vi "parse tdms properties_extract_priv_method.vi"(10 "property names":string[](array[string]), 11 "property values":variant[](array[variant])) -> (2 "channel units":string, 3 "nominal-compatible properties":map{string, string}(c390))   [LabVIEW 2020, in "Nominal-TDMS-Upload.lvlib" / "Nominal-TDMS-Upload.lvclass"]
uses:
  Nominal-TDMS-Upload.lvclass
  <vilib>/Nominal/Nominal IO Client/lv_src/Nominal Client/Nominal Client.lvclass
  <vilib>/Utility/Data Type/NI_Data Type.lvlib
  bb066b67-f704-4680-a74d-5f147d6b3788.vi
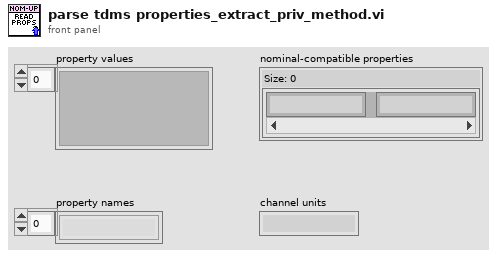
[diagram p1: front panel]
types:
  T1 = typedef "NI_Data Type.lvlib/Data Type.ctl" = enum8{"Invalid Type", "Void", "I8", "I16", "I32", "I64", "U8", "U16", "U32", "U64", "Single Float", "Double Float", "Extended Float", "Single Complex", "Double Complex", "Extended Complex", "Enum U8", "Enum U16", "Enum U32", "Enum U64", "Single Float With Unit", "Double Float With Unit", "Extended Float With Unit", "Single Complex with Unit", "Double Complex with Unit", "Extended Complex with Unit", "Boolean", "String", "Path", "Picture", "Tag", "Array", "Cluster", "Variant", "LV Variant", "Waveform", "Timestamp", "Digital Waveform", "Digital Data", "ExpressData", "Refnum", "External Data", "VI", "Poly VI", "LabVIEW Class Instance", "Fixed Point", "Set Collection", "Map Collection"}
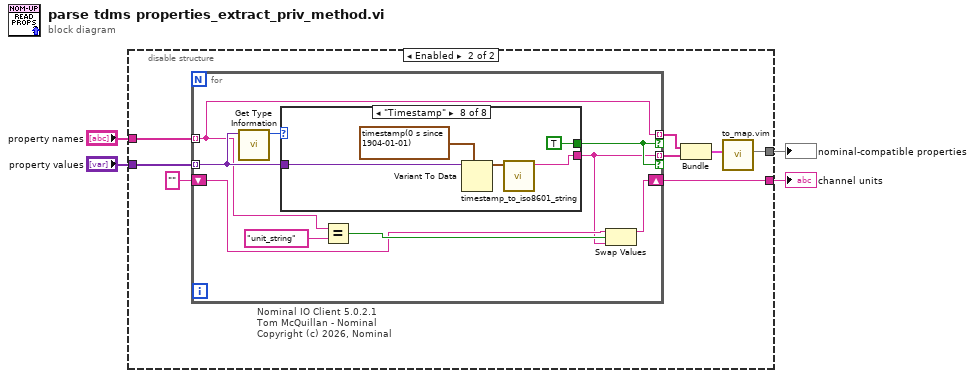
[diagram p0: block diagram]
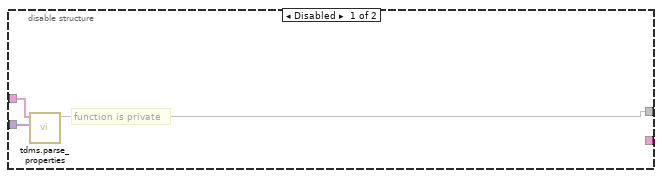
[diagram p2: hidden frame]
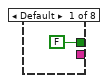
[diagram p3: hidden frame]
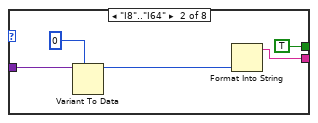
[diagram p4: hidden frame]
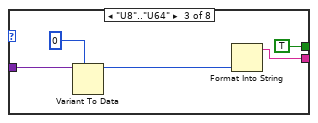
[diagram p5: hidden frame]
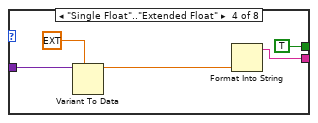
[diagram p6: hidden frame]
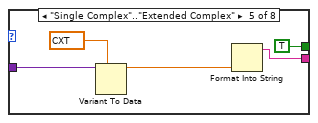
[diagram p7: hidden frame]
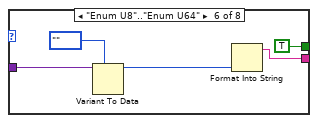
[diagram p8: hidden frame]
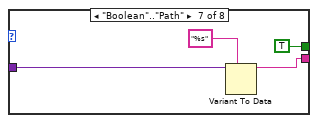
[diagram p9: hidden frame]
diagram:
  n1 = disable-structure shown="Enabled" {
    disable-tunnel: [w7 w10] -> w1
    disable-tunnel: "property names" -> [w6 w11]
    disable-tunnel: "property values" -> [w5 w12]
    disable-tunnel: [_ w8] -> w4
    frame Disabled {
      # "function is private"
      n2 = call <vilib>:"tdms.parse_properties.vi"("Property Values"=w5, "Property Names"=w6) -> ("Property Map"=w7:map{string, string})  [unwired: 9 in]
    }
    frame Enabled {
      # "Nominal IO Client 5.0.2.1\nTom McQuillan - Nominal\nCopyright (c) 2026, Nominal"
      n3 = for {
        tunnel: w12 -> [w23] mode=indexing
        tunnel: [w16] -> w15 mode=indexing if=w22
        tunnel: w11 -> [w21] mode=indexing
        tunnel: [w21] -> w14 mode=indexing if=w22
        shift-right: [w17] -> w8
        shift-left: "" -> [w18]
        n4 = call <vilib>:"Get Type Information.vi"("variant"=w23) -> ("type"=w24:T1)  [unwired: 6 in, 4 out]
        n5 = case shown="\"Timestamp\"" w24 {
          tunnel: w23 -> [_ w30 w35 w38 w43 w49 w54 w59]
          tunnel: [_ w27 w32 w37 w42 w47 w52 w55] -> w16
          tunnel: [FALSE TRUE TRUE TRUE TRUE TRUE TRUE TRUE] -> w22
          frame Default {
          }
          frame "I8".."I64" {
            n6 = Variant To Data(type=i64 0, Variant=w30) -> (data=w28:i64)  [unwired: 1 in, 1 out]
            n7 = Format Into String(w28) -> (resulting string=w27:string)  [unwired: 3 in, 1 out]
          }
          frame "U8".."U64" {
            n8 = Variant To Data(type=u64 0, Variant=w35) -> (data=w33:u64)  [unwired: 1 in, 1 out]
            n9 = Format Into String(w33) -> (resulting string=w32:string)  [unwired: 3 in, 1 out]
          }
          frame "Single Float".."Extended Float" {
            n10 = Variant To Data(type=ext 0.0, Variant=w38) -> (data=w39:ext)  [unwired: 1 in, 1 out]
            n11 = Format Into String(w39) -> (resulting string=w37:string)  [unwired: 3 in, 1 out]
          }
          frame "Single Complex".."Extended Complex" {
            n12 = Variant To Data(type=cxt 0.0+0.0i, Variant=w43) -> (data=w44:cxt)  [unwired: 1 in, 1 out]
            n13 = Format Into String(w44) -> (resulting string=w42:string)  [unwired: 3 in, 1 out]
          }
          frame "Enum U8".."Enum U64" {
            n14 = Variant To Data(type=enum32{""}."", Variant=w49) -> (data=w50:enum32{""})  [unwired: 1 in, 1 out]
            n15 = Format Into String(w50) -> (resulting string=w47:string)  [unwired: 3 in, 1 out]
          }
          frame "Boolean".."Path" {
            n16 = Variant To Data(type="%s", Variant=w54) -> (data=w52:string)  [unwired: 1 in, 1 out]
          }
          frame "Timestamp" {
            n17 = Variant To Data(type=timestamp(0 s since 1904-01-01), Variant=w59) -> (data=w56:timestamp)  [unwired: 1 in, 1 out]
            n18 = call <vilib>:"timestamp_to_iso8601_string.vi"("Time Stamp (now)"=w56) -> ("ISO8601 UTC DateTime"=w55:string)  [unwired: 10 in]
          }
        }
        n19 = Equal?(x=w21, y="unit_string") -> (x = y?=w19:bool)
        n20 = Swap Values(12:w18, 13:w19, 14:w16) -> (1:w17:string)  [unwired: 1 out]
      }
      n21 = Bundle(w14, w15) -> (w13:cluster{string[], string[]})  [unwired: 1 in]
      n22 = call "to_map.vim"("Map"=w13) -> ("Map out"=w10:map{string, string})  [unwired: 10 in]
    }
  }
  "channel units" <- w4
  "nominal-compatible properties" <- w1
